vi "Clear I2C Messages Table.vi"(5 "# TXNS IN TABLE Ref":refnum<vi>, 7 "I2C Table Ref":refnum<vi>, 8 "error in (no error)":errorcluster, 11 "Measurement UI Queue":refnum<queue>) -> (0 "error out":errorcluster)   [LabVIEW 2025, in "I2C Bus Monitor UI.lvlib"]
uses:
  I2C Bus Monitor UI.lvlib
  Table Buffer - Flush.vi
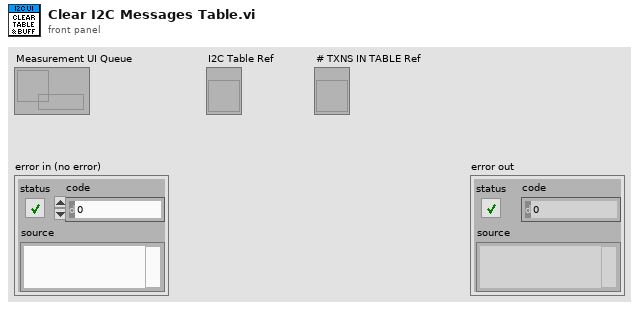
[diagram p1: front panel]
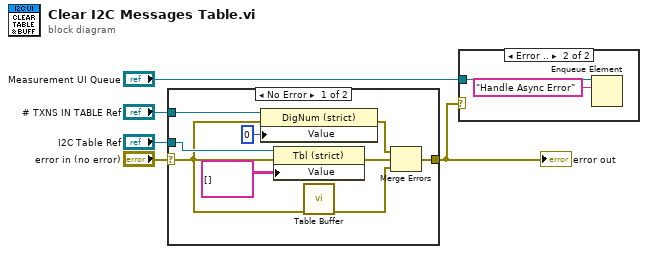
[diagram p0: block diagram]
diagram:
  n1 = case shown="No Error" "error in (no error)" {
    selector: "error in (no error)" -> [w11 w15]
    tunnel: "I2C Table Ref" -> [w14 _]
    tunnel: [w6 w15] -> w2
    tunnel: "# TXNS IN TABLE Ref" -> [w12 _]
    frame No Error {
      n2 = property on="Property Node" class="DigNum (strict)"(reference=w12, error in=w11, "Value"=0) -> (error out=w8:errorcluster)  [unwired: 1 out]
      n3 = property on="Property Node" class="Tbl (strict)"(reference=w14, error in=w11, "Value"=string[][] []) -> (error out=w9:errorcluster)  [unwired: 1 out]
      n4 = call-poly "Table Buffer.vi"("error in (no error)"=w11) -> ("error out"=w7:errorcluster)  [unwired: 10 in]
      n5 = Merge Errors(w8, w9, w7) -> (w6:errorcluster)
    }
    frame Error {
    }
  }
  "error out" <- w2
  n6 = case shown="Error .." w2 {
    tunnel: "Measurement UI Queue" -> [_ w17]
    frame No Error {
    }
    frame Error {
      n7 = Enqueue Element(queue=w17, element="Handle Async Error") -> ()  [unwired: 2 in, 3 out]
    }
  }
